vi "Parse Interface.vi"(8 "error in (no error)":errorcluster, 11 "Interface":string) -> (0 "error out":errorcluster, 2 "channel":u8, 3 "host":string)   [LabVIEW 2021, in "CAN RW CANsub.lvclass"]
uses:
  CAN RW CANsub.lvclass
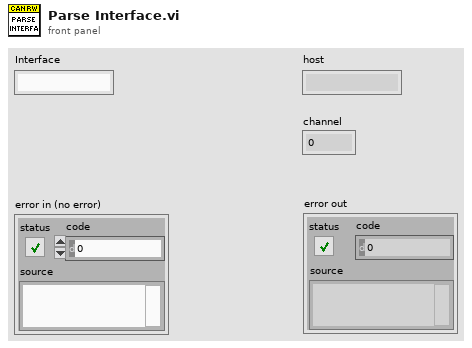
[diagram p1: front panel]
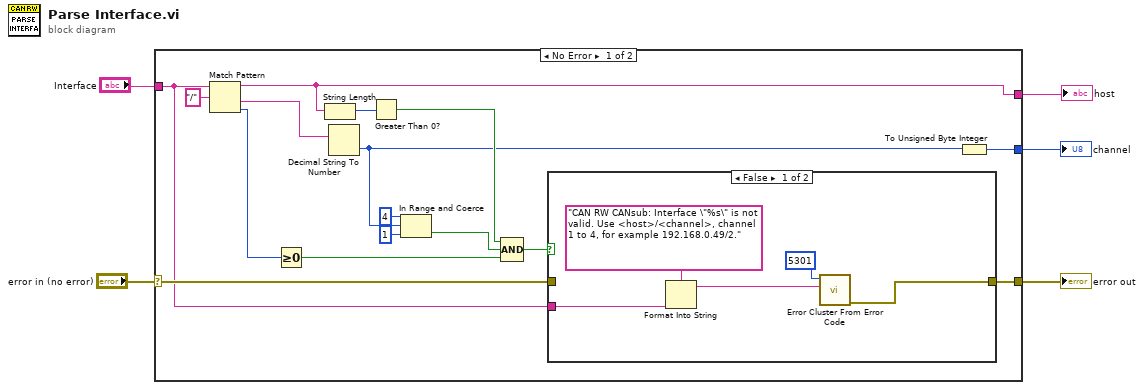
[diagram p0: block diagram]
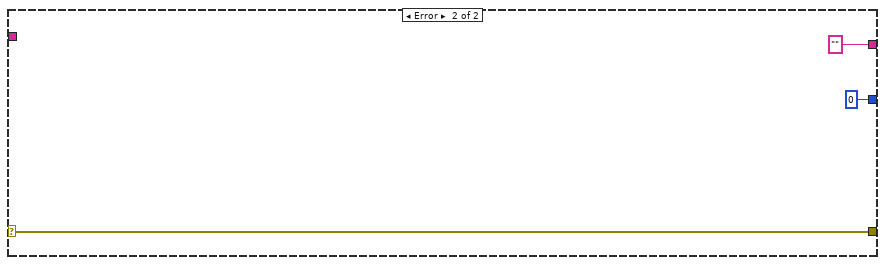
[diagram p3: hidden frame]
diagram:
  n1 = case shown="No Error" "error in (no error)" {
    selector: "error in (no error)" -> [w10 w30]
    tunnel: [w11 w30] -> w4
    tunnel: [w8 u8 0 ("channel")] -> w3
    tunnel: [w9 "" ("host")] -> w2
    tunnel: "Interface" -> [w6 _]
    frame No Error {
      n2 = Match Pattern(string=w6, regular expression="/") -> (before substring=w9:string, after substring=w20:string, offset past match=w19:i32)  [unwired: 1 in, 1 out]
      n3 = Greater Or Equal To 0?(x=w19) -> (x >= 0?=w12:bool)
      n4 = String Length(string=w9) -> (length=w18:i32)
      n5 = Decimal String To Number(string=w20) -> (number=w7:i32)  [unwired: 2 in, 1 out]
      n6 = Greater Than 0?(x=w18) -> (x > 0?=w15:bool)
      n7 = In Range and Coerce(upper limit=4, x=w7, lower limit=1) -> (In Range?=w13:bool)  [unwired: 1 out]
      n8 = Compound Arithmetic op=AND(w15, w13, w12) -> (w14:bool)
      n9 = case shown="False" w14 {
        tunnel: [w22 w27] -> w11
        tunnel: w10 -> [_ w27]
        tunnel: w6 -> [w25 _]
        frame False {
          n10 = Format Into String(format string="CAN RW CANsub: Interface \"%s\" is not valid. Use <host>/<channel>, channel 1 to 4, for example 192.168.0.49/2.", w25) -> (resulting string=w24:string)  [unwired: 2 in, 1 out]
          n11 = call <vilib>:"Error Cluster From Error Code.vi"("error message (\"\")"=w24, "error code (0)"=5301) -> ("error out"=w22:errorcluster)  [unwired: 7 in]
        }
        frame True {
        }
      }
      n12 = To Unsigned Byte Integer(number=w7) -> (unsigned 8bit integer=w8:u8)
    }
    frame Error {
    }
  }
  "host" <- w2
  "channel" <- w3
  "error out" <- w4
